vi "VIH HelpGen - Settings - Get Program for File Type.vi"(9 "EditPrograms":T1(array[cluster]), 11 "File Path":path) -> (0 "Found":bool, 1 "Program Path":path, 3 "dup File Path":path)   [LabVIEW 2014]
doc: "::: VI Helpeks :::\nCopyright (c) 2000-2026 Konstantin Shifershteyn. All rights reserved."
panel:
  # "VI Helpeks\nCopyright (c) 2012-2026 Konstantin Shifershteyn"
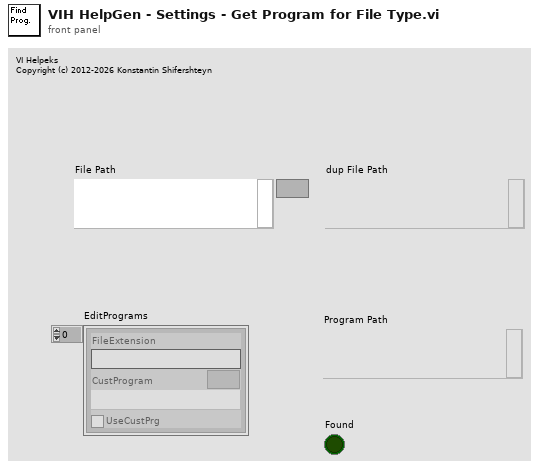
[diagram p1: front panel]
types:
  T1 = cluster{"FileExtension":string, "CustProgram":path, "UseCustPrg":bool}[]
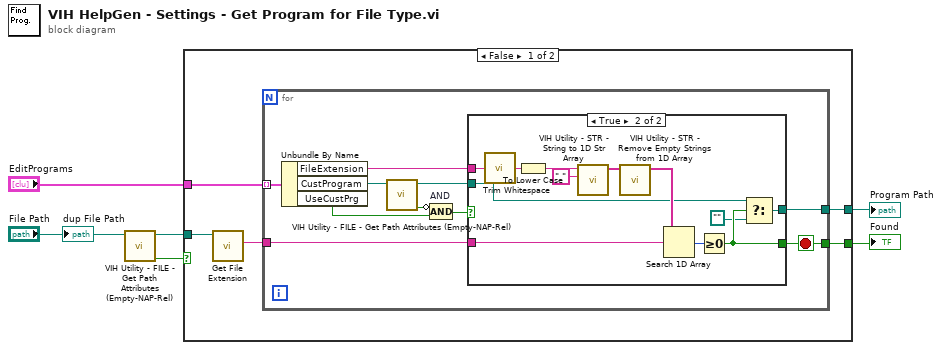
[diagram p0: block diagram]
diagram:
  n1 = call "VIH Utility - FILE - Get Path Attributes (Empty-NAP-Rel).vi"("Path"="File Path") -> ("Not A Path or Empty path"=w1:bool, "dup Path"=w2:path)  [unwired: 6 in, 3 out]
  n2 = case shown="False" w1 {
    tunnel: "EditPrograms" -> [w11 _]
    tunnel: [w9 _] -> w5
    tunnel: [w8 _] -> w4
    tunnel: w2 -> [w7 _]
    frame False {
      n3 = call <vilib>:"Get File Extension.vi"("file"=w7) -> ("lowercase file extension"=w10:string)  [unwired: 7 in, 3 out]
      n4 = for {
        tunnel: w11 -> [w21] mode=indexing
        tunnel: w10 -> [w15]
        tunnel: [w13] -> w9
        tunnel: [w12] -> w8
        stop <- w12 stop-if-true
        n5 = Unbundle By Name(w21) -> ("FileExtension"=w20:string, "CustProgram"=w19:path, "UseCustPrg"=w17:bool)
        n6 = call "VIH Utility - FILE - Get Path Attributes (Empty-NAP-Rel).vi"("Path"=w19) -> ("Not A Path or Empty path"=w18:bool, "dup Path"=w14:path)  [unwired: 6 in, 3 out]
        n7 = Compound Arithmetic op=AND "AND"(invert w18, w17) -> (w16:bool)
        n8 = case shown="True" w16 {
          tunnel: w20 -> [_ w33]
          tunnel: w15 -> [_ w28]
          tunnel: [_ w24] -> w12
          tunnel: w14 -> [_ w25]
          tunnel: [_ w22] -> w13
          frame False {
          }
          frame True {
            n9 = call <vilib>:"Trim Whitespace.vi"("string"=w33) -> ("trimmed string"=w32:string)  [unwired: 1 in]
            n10 = To Lower Case(string=w32) -> (all lower case string=w29:string)
            n11 = call "VIH Utility - STR - String to 1D Str Array.vi"("delimiter ('\\n')"=" " ("delimiter ('\\n')"), "String in"=w29) -> ("Array out"=w30:string[])  [unwired: 5 in]
            n12 = call "VIH Utility - STR - Remove Empty Strings from 1D Array.vi"("String array in"=w30) -> ("String array out"=w27:string[])  [unwired: 9 in, 1 out]
            n13 = Search 1D Array(1D array=w27, element=w28) -> (index of element=w26:i32)  [unwired: 1 in]
            n14 = Greater Or Equal To 0?(x=w26) -> (x >= 0?=w24:bool)
            n15 = Select(t=w25, s=w24, f=path "") -> (s? t:f=w22:path)
          }
        }
      }
    }
    frame True {
    }
  }
  "Program Path" <- w5
  "Found" <- w4
  "dup File Path" <- "File Path"
